vi "Main Page.vi"(8 "error in (no error)":errorcluster, 11 "Node Ptr":T11 format="%.0x") -> (0 "error out":errorcluster)   [LabVIEW 2020, in "NI Synchronization System Explorer.lvlib"]
uses:
  NI Synchronization System Explorer.lvlib
  <vilib>/NI VeriStand/Custom Device API/Custom Device Item Ref.ctl
  Connection Selection.ctl
  Shared/Routes.ctl
  Shared/Route.ctl
  Pins Tab.ctl
  Shared/Mode.ctl
  Shared/External Pin.ctl
  Shared/Time Reference.ctl
  Time Ref Tab.ctl
  Shared/IRIG Type.ctl
  Shared/Constants.vi
  <vilib>/NI VeriStand/Custom Device API/Get Item Property (Boolean).vi
  sub_EnableDisable Control.vi
  <vilib>/NI VeriStand/Custom Device API/Get Item Property (String).vi
  <vilib>/NI VeriStand/Custom Device API/Get Item Property (U16).vi
  <vilib>/NI VeriStand/Custom Device API/Get Item Property (Double).vi
  <vilib>/NI VeriStand/Custom Device API/Set Item Property (String).vi
  <vilib>/NI VeriStand/Custom Device API/Set Item Property (Boolean).vi
  <vilib>/NI VeriStand/Custom Device API/Set Item Property (Variant).vi
  <vilib>/NI VeriStand/Custom Device API/Set Item Property (U16).vi
  <vilib>/NI VeriStand/Custom Device API/Set Item Property (I32).vi
  <vilib>/NI VeriStand/Custom Device API/Set Item Property (Double).vi
  <vilib>/NI VeriStand/Custom Device API/Custom Device API.lvlib
  Shared/NI Synchronization Shared.lvlib
panel:
  in  "6683H Warning":string
  in  "SyncModule":string caption="Chassis Clock Generation Module"
  in  "SyncModule?":bool
  in  "Settings":T1(tab)
  out "TimeRefTab":T2
  in  "Priority 2":i32 min=0 max=255
  in  "Priority 1":i32 min=0 max=255
  in  "IRIG type":T3=enum."IRIGB AM"
  in  "Start Time":timestamp
  in  "PPSSetTime":bool
  in  "Terminal":string
  in  "Time Reference":T4
  out "Mode Desciption 2":string="When using a time reference other than PXI Chassis Clock, it is recommended to additionally configure that time reference in Measurement and Automation Explorer (MAX) before deployment. Doing so will prevent \"macro\" adjustments to system time while the NI VeriStand engine is running."
  out "Mode Desciption":string
  in  "Mode":T5
  in  "ConSelection":T6 caption="Selection"
  out "Pins tab":T7
  in  "PFI2":bool
  in  "PFI1":bool
  in  "PFI0":bool
  in  "PXI_Trig0":bool
  in  "Route In Pin":T8
  in  "Custom Routes":T9
  in  "StartDelay":u16 caption="Generation Start Delay (s)"
  in  "PhaseOffset":dbl caption="Generation Phase Offset (°)" min=0.0 max=360.0
  in  "timekeeper":string caption="Time-Based Synchronization Module"
  in  "Header":cluster{"Section Name":string}={"Section Name"="NI Synchronization Settings"}
  in  "Description":string
  in  "Name":string
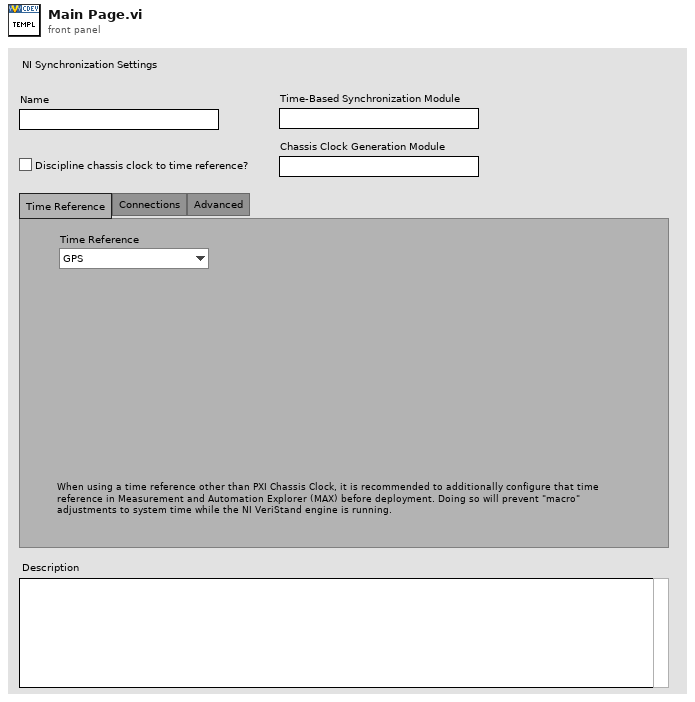
[diagram p1: front panel]
types:
  T1 = enum32{"Time Reference", "Connections", "Advanced"}
  T2 = typedef "NI Synchronization System Explorer.lvlib/Time Ref Tab.ctl" = enum32{"Empty", "1588", "IRIG", "PPS"}
  T3 = typedef "NI Synchronization Shared.lvlib/IRIG Type.ctl" = enum16{"IRIGB DC", "IRIGB AM"}
  T4 = typedef "NI Synchronization Shared.lvlib/Time Reference.ctl" = enum16{"GPS", "IRIG", "PPS", "1588 Ordinary Clock", "802.1AS", "PXI Chassis Clock", "Free Running (Internal)"}
  T5 = typedef "NI Synchronization Shared.lvlib/Mode.ctl" = enum16{"Generate sample clock", "Route sample clock out of chassis", "Route sample clock into chassis", "Custom routes"}
  T6 = typedef "NI Synchronization System Explorer.lvlib/Connection Selection.ctl" = enum16{"Automatic", "Custom"}
  T7 = typedef "NI Synchronization System Explorer.lvlib/Pins Tab.ctl" = enum32{"Pins", "Ext. Pin", "Custom"}
  T8 = typedef "NI Synchronization Shared.lvlib/External Pin.ctl" = enum16{"PFI0", "PFI1", "PFI2"}
  T9 = typedef "NI Synchronization Shared.lvlib/Routes.ctl" = T10[]
  T10 = typedef "NI Synchronization Shared.lvlib/Route.ctl" = cluster{"Source":string, "Destination":string}
  T11 = typedef "Custom Device API.lvlib/Custom Device Item Ref.ctl" = u64
  T12 = typedef "NI Synchronization Shared.lvlib/Connection Settings.ctl" = cluster{"Mode":T5, "pxitrig":bool, "pfi0":bool, "pfi1":bool, "pfi2":bool, "External Pin":T8, "Routes":T9}
  T13 = typedef "Custom Device API.lvlib/Custom Device Item Info.ctl" = cluster{"Name":string, "Is Channel":bool, "GUID":string, "Is Waveform":bool}
  T14 = typedef "NI Synchronization Shared.lvlib/Time Ref Settings.ctl" = cluster{"Time Reference":T4, "Priority 1":i32, "Priority 2":i32, "IRIG type":T3, "Terminal":string, "PPSSetTime":bool, "Start Time":timestamp}
  T15 = typedef "Custom Device API.lvlib/Custom Device Commands.ctl" = enum16{"Default", "Item renamed", "Shutdown", "Dynamic button pressed"}
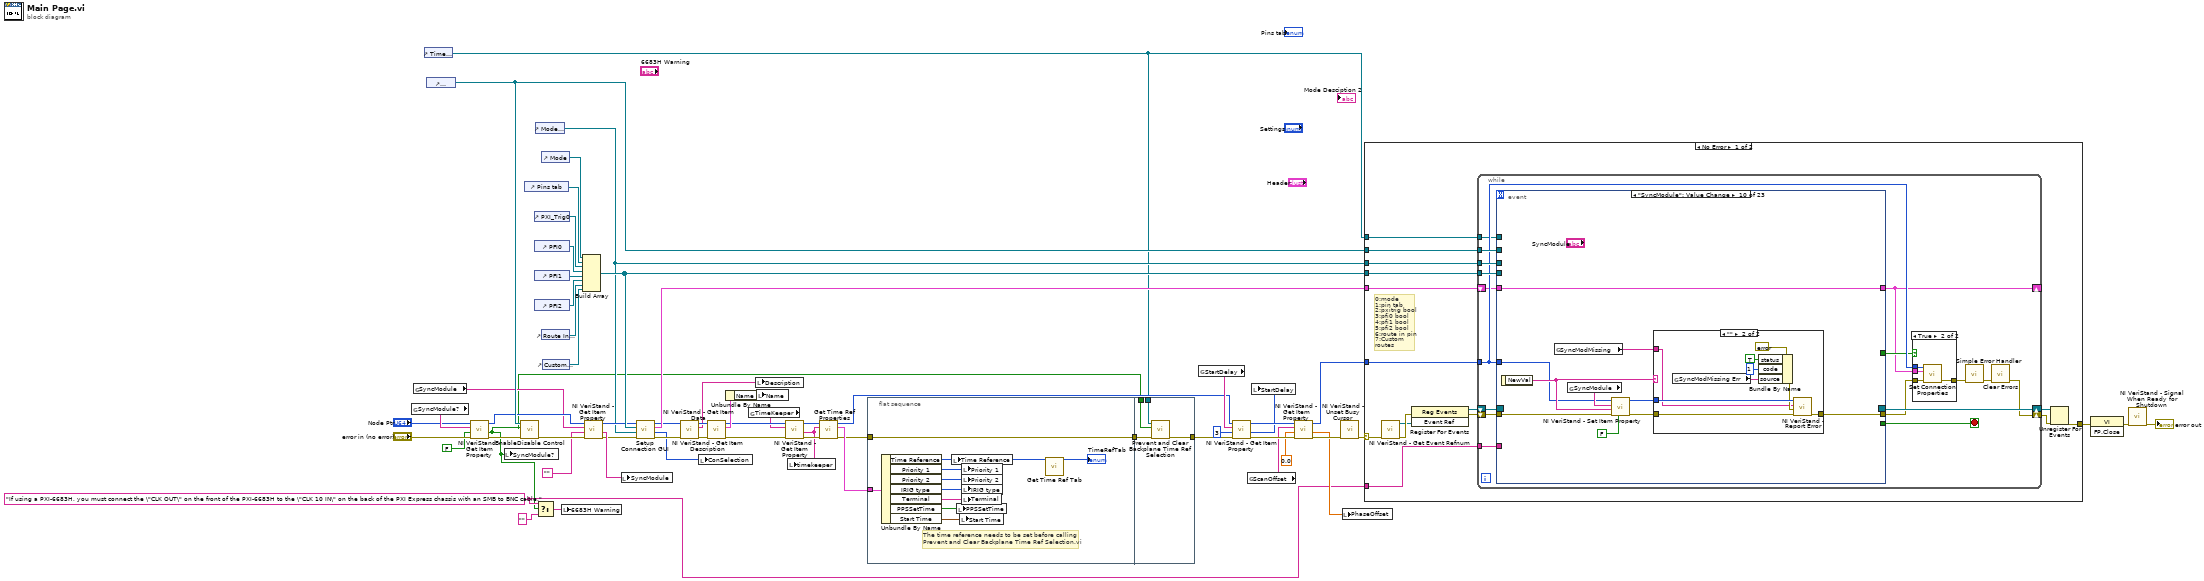
[diagram p0: block diagram]
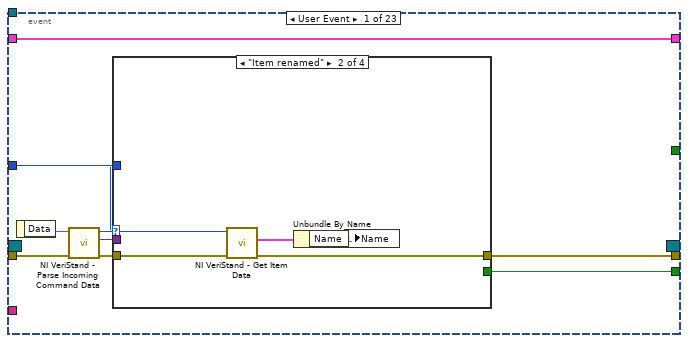
[diagram p3: hidden frame]
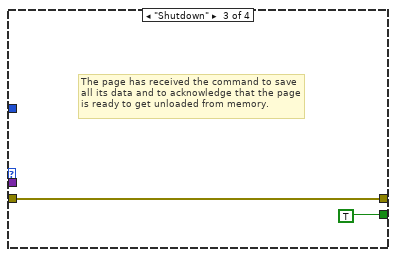
[diagram p5: hidden frame]
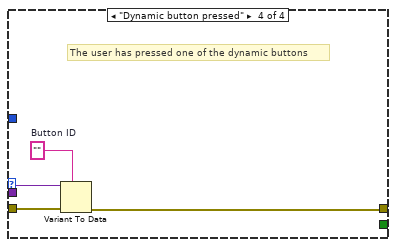
[diagram p6: hidden frame]
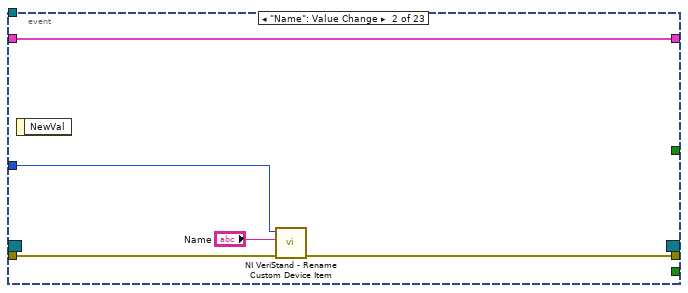
[diagram p7: hidden frame]
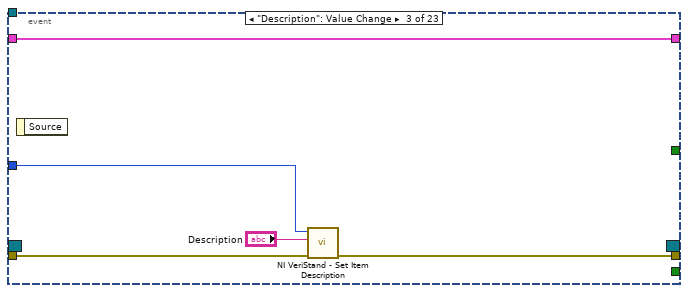
[diagram p8: hidden frame]
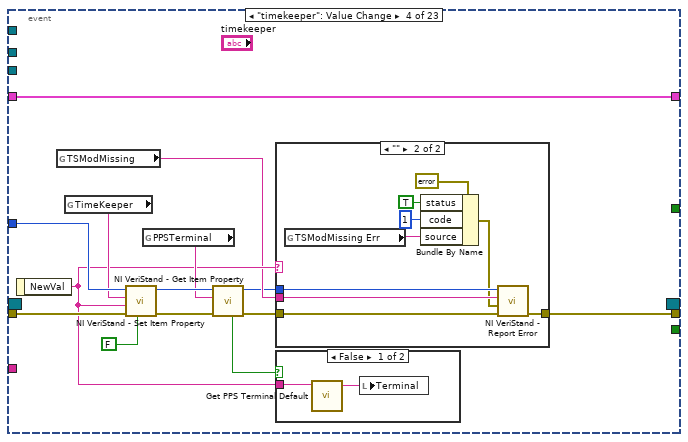
[diagram p9: hidden frame]
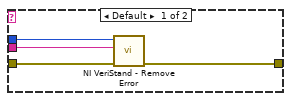
[diagram p10: hidden frame]
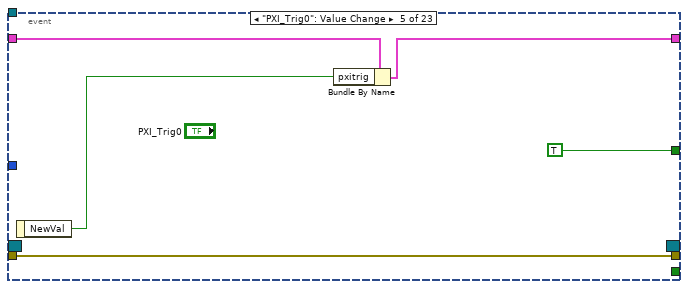
[diagram p12: hidden frame]
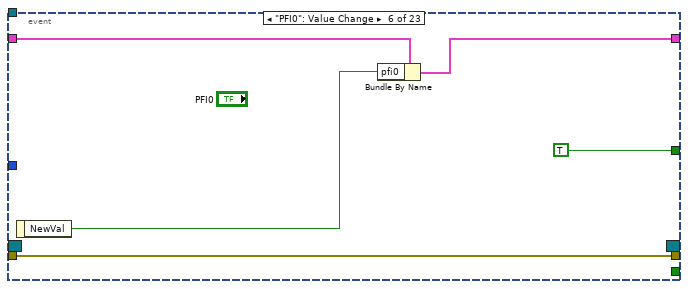
[diagram p13: hidden frame]
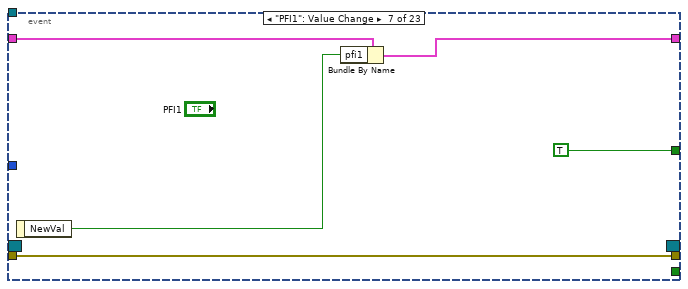
[diagram p14: hidden frame]
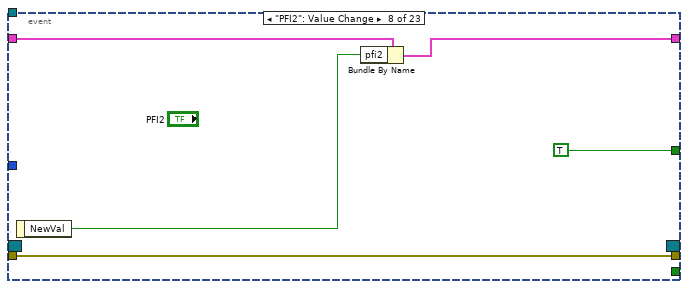
[diagram p15: hidden frame]
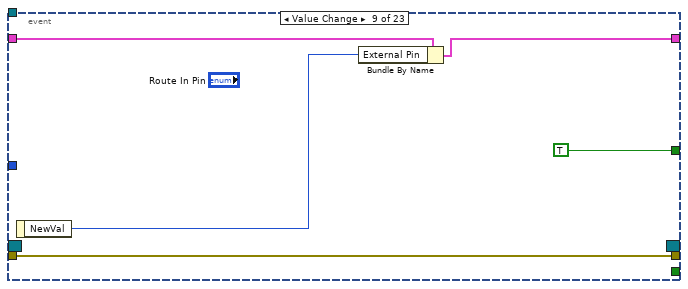
[diagram p16: hidden frame]
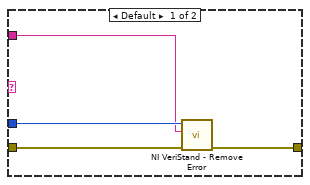
[diagram p17: hidden frame]
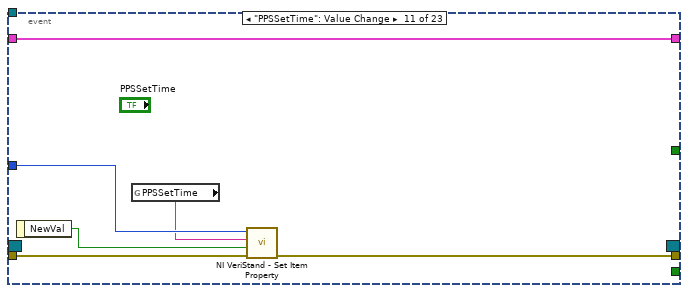
[diagram p18: hidden frame]
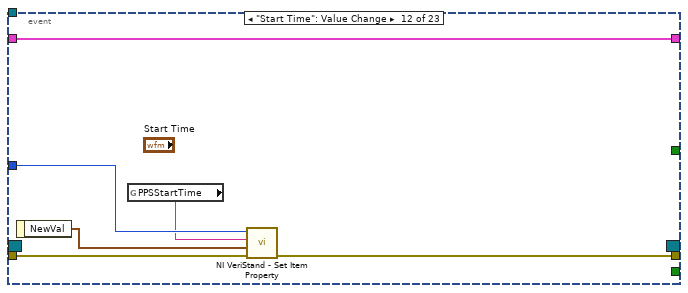
[diagram p19: hidden frame]
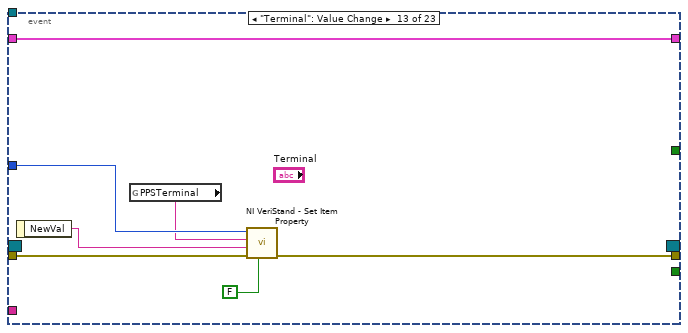
[diagram p20: hidden frame]
diagram:
  w7 = "If using a PXI-6683H, you must connect the \"CLK OUT\" on the front of the PXI-6683H to the \"CLK 10 IN\" on the back of the PXI Express chassis with an SMB to BNC cable." ("6683H Warning")
  n1 = global read "Constants.vi" "SyncModule?"() -> (w27:string)
  n2 = global read "Constants.vi" "SyncModule"() -> (w22:string)
  n3 = control-ref of="Time Reference"() -> (w2:refnum<vi>)
  n4 = control-ref of="SyncModule"() -> (w24:refnum<vi>)
  n5 = call-poly <vilib>:"NI VeriStand - Get Item Property.vi"("error in (no error)"="error in (no error)", "Default Value"=FALSE, "Property Name"=w27, "Item Ref in"="Node Ptr") -> ("error out"=w28:errorcluster, "Value"=w1:bool, "Item Ref out"=w23:T11)  [unwired: 4 in, 1 out]
  n6 = local write "SyncModule?"(w1) -> ()
  n7 = call-poly "EnableDisable Control.vi"("error in (no error)"=w28, "Enable"=w1, "Control"=w24) -> ("error out"=w25:errorcluster)  [unwired: 8 in]
  n8 = control-ref of="Pins tab"() -> (w38:refnum<vi>)
  n9 = control-ref of="PXI_Trig0"() -> (w37:refnum<vi>)
  n10 = control-ref of="PFI0"() -> (w36:refnum<vi>)
  n11 = control-ref of="PFI1"() -> (w31:refnum<vi>)
  n12 = control-ref of="PFI2"() -> (w32:refnum<vi>)
  n13 = control-ref of="Mode Desciption"() -> (w12:refnum<vi>)
  n14 = Select(t=w7, s=w1, f="" ("6683H Warning")) -> (s? t:f=w8:string)
  n15 = control-ref of="Mode"() -> (w39:refnum<vi>)
  n16 = control-ref of="Route In Pin"() -> (w35:refnum<vi>)
  n17 = control-ref of="Custom Routes"() -> (w34:refnum<vi>)
  n18 = local write "6683H Warning"(w8) -> ()
  n19 = Build Array(w39, w38, w37, w36, w31, w32, w35, w34) -> (w29:refnum<vi>[])
  n20 = call-poly <vilib>:"NI VeriStand - Get Item Property.vi"("error in (no error)"=w25, "Default Value"="", "Property Name"=w22, "Item Ref in"=w23) -> ("error out"=w10:errorcluster, "Value"=w20:string, "Item Ref out"=w13:T11)  [unwired: 4 in, 1 out]
  n21 = local write "SyncModule"(w20) -> ()
  n22 = call "Setup Connection GUI.vi"("error in (no error)"=w10, "Mode Description Control"=w12, "Connection Controls"=w29, "Item Ref in"=w13) -> ("error out"=w30:errorcluster, "ConSelection"=w16:T6, "Connection Settings"=w15:T12, "Item Ref out"=w14:T11)  [unwired: 4 in]
  n23 = call <vilib>:"NI VeriStand - Get Item Description.vi"("error in (no error)"=w30, "Item Ref in"=w14) -> ("error out"=w56:errorcluster, "Description"=w57:string, "Item Ref out"=w58:T11)  [unwired: 7 out]
  n24 = local write "ConSelection"(w16) -> ()
  n25 = call <vilib>:"NI VeriStand - Get Item Data.vi"("error in (no error)"=w56, "Item Ref in"=w58) -> ("error out"=w53:errorcluster, "Item Info"=w55:T13, "Item Ref out"=w52:T11)  [unwired: 7 out]
  n26 = Unbundle By Name(w55) -> ("Name"=w54:string)
  n27 = global read "Constants.vi" "TimeKeeper"() -> (w51:string)
  n28 = local write "Description"(w57) -> ()
  n29 = local write "Name"(w54) -> ()
  n30 = call-poly <vilib>:"NI VeriStand - Get Item Property.vi"("error in (no error)"=w53, "Property Name"=w51, "Item Ref in"=w52) -> ("error out"=w50:errorcluster, "Value"=w18:string, "Item Ref out"=w19:T11)  [unwired: 5 in, 1 out]
  n31 = local write "timekeeper"(w18) -> ()
  n32 = call "Get Time Ref Properties.vi"("error in (no error)"=w50, "TimeKeeper Module"=w18, "Device Item Ref in"=w19) -> ("error out"=w6:errorcluster, "Time Ref Settings"=w17:T14, "Item Ref out"=w4:T11)  [unwired: 6 in]
  n33 = flat-sequence {
    tunnel: w17 -> [w72]
    tunnel: w6 -> [w63]
    tunnel: [w63] -> w3
    tunnel: [w75] -> w5
    tunnel: w3 -> [w76]
    tunnel: w2 -> [w74]
    tunnel: w1 -> [w73]
    frame #0 {
      # "The time reference needs to be set before calling \nPrevent and Clear Backplane Time Ref Selection.vi"
      n34 = Unbundle By Name(w72) -> ("Time Reference"=w65:T4, "Priority 1"=w71:i32, "Priority 2"=w70:i32, "IRIG type"=w69:T3, "Terminal"=w68:string, "PPSSetTime"=w67:bool, "Start Time"=w66:timestamp)
      n35 = local write "Time Reference"(w65) -> ()
      n36 = local write "PPSSetTime"(w67) -> ()
      n37 = local write "Start Time"(w66) -> ()
      n38 = local write "Priority 1"(w71) -> ()
      n39 = local write "Priority 2"(w70) -> ()
      n40 = local write "IRIG type"(w69) -> ()
      n41 = local write "Terminal"(w68) -> ()
      n42 = call "Get Time Ref Tab.vi"("Time Ref"=w65) -> ("TimeRefTab"=→"TimeRefTab":T2)  [unwired: 10 in]
    }
    frame #1 {
      n43 = call "Prevent and Clear Backplane Time Ref Selection.vi"("error in (no error)"=w76, "Sync Mod?"=w73, "Time Reference Enum"=w74) -> ("error out"=w75:errorcluster)  [unwired: 8 in]
    }
  }
  n44 = global read "Constants.vi" "StartDelay"() -> (w45:string)
  n45 = call-poly <vilib>:"NI VeriStand - Get Item Property.vi"("error in (no error)"=w5, "Default Value"=u16 3 ("Start Offset Multiple"), "Property Name"=w45, "Item Ref in"=w4) -> ("error out"=w46:errorcluster, "Value"=w43:u16, "Item Ref out"=w49:T11)  [unwired: 4 in, 1 out]
  n46 = global read "Constants.vi" "ScanOffset"() -> (w42:string)
  n47 = local write "StartDelay"(w43) -> ()
  n48 = call-poly <vilib>:"NI VeriStand - Get Item Property.vi"("error in (no error)"=w46, "Default Value"=0.0 ("Scan Offset Scale (%)"), "Property Name"=w42, "Item Ref in"=w49) -> ("error out"=w47:errorcluster, "Value"=w40:dbl, "Item Ref out"=w48:T11)  [unwired: 4 in, 1 out]
  n49 = call <vilib>:"NI VeriStand - Unset Busy Cursor.vi"("error in (no error)"=w47) -> ("error out"=w59:errorcluster)  [unwired: 10 out]
  n50 = local write "PhaseOffset"(w40) -> ()
  n51 = case shown="No Error" w59 {
    selector: w59 -> [w83 w357]
    tunnel: [w88 w355] -> w62
    tunnel: w48 -> [w84 _]
    tunnel: w29 -> [w82 _]
    tunnel: w12 -> [w81 _]
    tunnel: w24 -> [w80 _]
    tunnel: w15 -> [w79 _]
    tunnel: w2 -> [w78 _]
    tunnel: w7 -> [w77 _]
    frame No Error {
      # "0:mode\n1:pin tab\n2:pxitrig bool\n3:pfi0 bool\n4:pfi1 bool\n5:pfi2 bool\n6:route in pin\n7:Custom routes"
      n52 = call <vilib>:"NI VeriStand - Get Event Refnum.vi"("error in (no error)"=w83) -> ("error out"=w91:errorcluster, "Event Ref"=w87:refnum<user-event>)  [unwired: 9 out]
      n53 = register-events(error in=w91, w87) -> (reference out=w85:refnum<event-registration>, error out=w86:errorcluster)  [unwired: 1 in]
      n54 = while {
        tunnel: w84 -> [w97]
        shift-right: [w103] -> w89
        shift-left: w86 -> [w107]
        shift-right: [w108] -> w90
        shift-left: w85 -> [w106]
        tunnel: w82 -> [w102]
        tunnel: w81 -> [w101]
        tunnel: w80 -> [w100]
        shift-right: [w93] -> _
        shift-left: w79 -> [w96]
        tunnel: w78 -> [w94]
        tunnel: w77 -> [w92]
        stop <- w105 stop-if-true
        n55 = event shown="[9] \"SyncModule\": Value Change" {
          selector: w106 -> [_ _ _ _ _ _ _ _ _ _ _ _ _ _ _ _ _ _ _ _ _ _ _]
          dyn-events: [_ _ _ _ _ _ _ _ _ _ _ _ _ _ _ _ _ _ _ _ _ _ _] -> w108
          timeout: _ -> [_ _ _ _ _ _ _ _ _ _ _ _ _ _ _ _ _ _ _ _ _ _ _]
          tunnel: w107 -> [w122 w139 w143 w158 w178 w183 w188 w193 w198 w208 w227 w233 w240 w247 w253 w259 w265 w284 w302 w308 w314 w327 w350]
          tunnel: [w118 _ _ _ _ _ _ _ _ _ _ _ _ _ _ _ _ _ _ _ _ _ _] -> w105
          tunnel: [w117 w138 w142 w147 w178 w183 w188 w193 w198 w201 w223 w229 w236 w244 w249 w255 w261 w272 w302 w304 w310 w322 w347] -> w98
          tunnel: w97 -> [w116 w137 w144 w157 _ _ _ _ _ w199 w226 w232 w239 w246 w252 w258 w264 w277 _ w307 w313 w326 _]
          tunnel: w102 -> [_ _ _ _ _ _ _ _ _ _ _ _ _ _ _ _ _ _ _ _ _ w324 w348]
          tunnel: w101 -> [_ _ _ _ _ _ _ _ _ _ _ _ _ _ _ _ _ _ _ _ _ w323 _]
          tunnel: w100 -> [_ _ _ _ _ _ _ _ _ _ _ _ _ _ _ _ _ w281 _ _ _ _ _]
          tunnel: [w114 w135 w140 w155 w175 w181 w186 w191 w196 w206 w222 w228 w235 w243 w248 w254 w260 w280 w300 w303 w309 w315 w336] -> w93
          tunnel: w96 -> [w114 w135 w140 w155 w176 w182 w187 w192 w197 w206 w222 w228 w235 w243 w248 w254 w260 w280 w301 w303 w309 w317 w337]
          tunnel: [_ _ _ _ TRUE TRUE TRUE TRUE TRUE _ _ _ _ _ _ _ _ _ TRUE _ _ _ TRUE] -> w95
          tunnel: w94 -> [_ _ _ _ _ _ _ _ _ _ _ _ _ _ _ _ _ w279 _ _ _ _ _]
          tunnel: w92 -> [_ _ _ _ _ _ _ _ _ _ _ _ _ _ _ _ _ w276 _ _ _ _ _]
          event User Event {
            n56 = event-data() -> ("Data"=w121:string)  [unwired: 1 out]
            n57 = call <vilib>:"NI VeriStand - Parse Incoming Command Data.vi"("error in (no error)"=w122, "Incoming data"=w121) -> ("error out"=w120:errorcluster, "Outgoing data"=w115:variant, "Action"=w119:T15)  [unwired: 7 out]
            n58 = case shown="\"Item renamed\"" w119 {
              tunnel: w120 -> [w123 w128 w129 w134]
              tunnel: [_ _ TRUE _] -> w118
              tunnel: [w123 w125 w129 w131] -> w117
              tunnel: w116 -> [_ w127 _ _]
              tunnel: w115 -> [_ _ _ w133]
              frame "Default", Default {
              }
              frame "Item renamed" {
                n59 = call <vilib>:"NI VeriStand - Get Item Data.vi"("error in (no error)"=w128, "Item Ref in"=w127) -> ("error out"=w125:errorcluster, "Item Info"=w126:T13)  [unwired: 8 out]
                n60 = Unbundle By Name(w126) -> ("Name"=w124:string)
                n61 = local write "Name"(w124) -> ()
              }
              frame "Shutdown" {
                # "The page has received the command to save all its data and to acknowledge that the page is ready to get unloaded from memory."
              }
              frame "Dynamic button pressed" {
                w132 = ""  # Button ID
                # "The user has pressed one of the dynamic buttons"
                n62 = Variant To Data(error in=w134, type=w132, Variant=w133) -> (error out=w131:errorcluster)  [unwired: 1 out]
              }
            }
          }
          event "Name": Value Change {
            n63 = event-data() -> ()  [unwired: 2 out]
            n64 = call <vilib>:"NI VeriStand - Rename Custom Device Item.vi"("error in (no error)"=w139, "New Name"="Name", "Item Ref in"=w137) -> ("error out"=w138:errorcluster)  [unwired: 1 in, 7 out]
          }
          event "Description": Value Change {
            n65 = event-data() -> ()  [unwired: 2 out]
            n66 = call <vilib>:"NI VeriStand - Set Item Description.vi"("error in (no error)"=w143, "Description"="Description", "Item Ref in"=w144) -> ("error out"=w142:errorcluster)  [unwired: 8 out]
          }
          event "timekeeper": Value Change {
            n67 = event-data() -> ("NewVal"=w148:string)  [unwired: 1 out]
            n68 = global read "Constants.vi" "TSModMissing"() -> (w146:string)
            n69 = global read "Constants.vi" "TimeKeeper"() -> (w156:string)
            n70 = call-poly <vilib>:"NI VeriStand - Set Item Property.vi"("Binary String (T)"=FALSE, "error in (no error)"=w158, "Value"=w148, "Property Name"=w156, "Item Ref in"=w157) -> ("error out"=w153:errorcluster, "Item Ref out"=w152:T11)  [unwired: 4 in, 1 out]
            n71 = global read "Constants.vi" "PPSTerminal"() -> (w151:string)
            n72 = call-poly <vilib>:"NI VeriStand - Get Item Property.vi"("error in (no error)"=w153, "Property Name"=w151, "Item Ref in"=w152) -> ("error out"=w149:errorcluster, "Item Ref out"=w145:T11, "Found?"=w150:bool)  [unwired: 5 in, 1 out]
            n73 = case shown="\"\"" w148 {
              tunnel: w149 -> [w162 w171]
              tunnel: [w159 w170] -> w147
              tunnel: w146 -> [w161 w169]
              tunnel: w145 -> [w160 w168]
              frame Default {
                n74 = call <vilib>:"NI VeriStand - Remove Error.vi"("error in (no error)"=w162, "Error ID"=w161, "Node Ref in"=w160) -> ("error out"=w159:errorcluster)  [unwired: 7 in, 1 out]
              }
              frame "" {
                n75 = global read "Constants.vi" "TSModMissing Err"() -> (w164:string)
                n76 = Bundle By Name(cluster=errorcluster {"status"=FALSE, "code"=0, "source"=""} ("error constant"), "status"=TRUE, "code"=1, "source"=w164) -> (w163:errorcluster)
                n77 = call <vilib>:"NI VeriStand - Report Error.vi"("error in (no error)"=w171, "New Error"=w163, "Error ID"=w169, "Node Ref in"=w168) -> ("error out"=w170:errorcluster)  [unwired: 6 in, 1 out]
              }
            }
            n78 = case shown="False" w150 {
              tunnel: w148 -> [w173 _]
              frame False {
                n79 = call "Get PPS Terminal Default.vi"("TimeKeeper Module"=w173) -> ("PPSTerminal Default"=w172:string)  [unwired: 10 in]
                n80 = local write "Terminal"(w172) -> ()
              }
              frame True {
              }
            }
          }
          event "PXI_Trig0": Value Change {
            n81 = event-data() -> ("NewVal"=w177:bool)  [unwired: 1 out]
            n82 = Bundle By Name(cluster=w176, "pxitrig"=w177) -> (w175:T12)
          }
          event "PFI0": Value Change {
            n83 = event-data() -> ("NewVal"=w180:bool)  [unwired: 1 out]
            n84 = Bundle By Name(cluster=w182, "pfi0"=w180) -> (w181:T12)
          }
          event "PFI1": Value Change {
            n85 = event-data() -> ("NewVal"=w185:bool)  [unwired: 1 out]
            n86 = Bundle By Name(cluster=w187, "pfi1"=w185) -> (w186:T12)
          }
          event "PFI2": Value Change {
            n87 = event-data() -> ("NewVal"=w190:bool)  [unwired: 1 out]
            n88 = Bundle By Name(cluster=w192, "pfi2"=w190) -> (w191:T12)
          }
          event Value Change {
            n89 = event-data() -> ("NewVal"=w195:T8)  [unwired: 1 out]
            n90 = Bundle By Name(cluster=w197, "External Pin"=w195) -> (w196:T12)
          }
          event "SyncModule": Value Change {
            n91 = event-data() -> ("NewVal"=w203:string)  [unwired: 1 out]
            n92 = global read "Constants.vi" "SyncModMissing"() -> (w200:string)
            n93 = global read "Constants.vi" "SyncModule"() -> (w207:string)
            n94 = call-poly <vilib>:"NI VeriStand - Set Item Property.vi"("Binary String (T)"=FALSE, "error in (no error)"=w208, "Value"=w203, "Property Name"=w207, "Item Ref in"=w199) -> ("error out"=w202:errorcluster, "Item Ref out"=w204:T11)  [unwired: 4 in, 1 out]
            n95 = case shown="\"\"" w203 {
              tunnel: w202 -> [w212 w221]
              tunnel: [w210 w220] -> w201
              tunnel: w204 -> [w211 w219]
              tunnel: w200 -> [w209 w213]
              frame Default {
                n96 = call <vilib>:"NI VeriStand - Remove Error.vi"("error in (no error)"=w212, "Error ID"=w209, "Node Ref in"=w211) -> ("error out"=w210:errorcluster)  [unwired: 7 in, 1 out]
              }
              frame "" {
                n97 = global read "Constants.vi" "SyncModMissing Err"() -> (w214:string)
                n98 = Bundle By Name(cluster=errorcluster {"status"=FALSE, "code"=0, "source"=""} ("error constant"), "status"=TRUE, "code"=1, "source"=w214) -> (w215:errorcluster)
                n99 = call <vilib>:"NI VeriStand - Report Error.vi"("error in (no error)"=w221, "New Error"=w215, "Error ID"=w213, "Node Ref in"=w219) -> ("error out"=w220:errorcluster)  [unwired: 6 in, 1 out]
              }
            }
          }
          event "PPSSetTime": Value Change {
            n100 = event-data() -> ("NewVal"=w224:bool)  [unwired: 1 out]
            n101 = global read "Constants.vi" "PPSSetTime"() -> (w225:string)
            n102 = call-poly <vilib>:"NI VeriStand - Set Item Property.vi"("error in (no error)"=w227, "Value"=w224, "Property Name"=w225, "Item Ref in"=w226) -> ("error out"=w223:errorcluster)  [unwired: 5 in, 2 out]
          }
          event "Start Time": Value Change {
            n103 = event-data() -> ("NewVal"=w230:timestamp)  [unwired: 1 out]
            n104 = global read "Constants.vi" "PPSStartTime"() -> (w231:string)
            n105 = call-poly <vilib>:"NI VeriStand - Set Item Property.vi"("error in (no error)"=w233, "Value"=w230, "Property Name"=w231, "Item Ref in"=w232) -> ("error out"=w229:errorcluster)  [unwired: 5 in, 2 out]
          }
          event "Terminal": Value Change {
            n106 = event-data() -> ("NewVal"=w237:string)  [unwired: 1 out]
            n107 = global read "Constants.vi" "PPSTerminal"() -> (w238:string)
            n108 = call-poly <vilib>:"NI VeriStand - Set Item Property.vi"("Binary String (T)"=FALSE, "error in (no error)"=w240, "Value"=w237, "Property Name"=w238, "Item Ref in"=w239) -> ("error out"=w236:errorcluster)  [unwired: 4 in, 2 out]
          }
          event Value Change {
            n109 = event-data() -> ("NewVal"=w242:T4)  [unwired: 1 out]
            n110 = call "Get Time Ref Tab.vi"("Time Ref"=w242) -> ("TimeRefTab"=w241:T2)  [unwired: 10 in]
            n111 = global read "Constants.vi" "TimeRef"() -> (w245:string)
            n112 = local write "TimeRefTab"(w241) -> ()
            n113 = call-poly <vilib>:"NI VeriStand - Set Item Property.vi"("error in (no error)"=w247, "Value"=w242, "Property Name"=w245, "Item Ref in"=w246) -> ("error out"=w244:errorcluster)  [unwired: 5 in, 2 out]
          }
          event Value Change {
            n114 = event-data() -> ("NewVal"=w250:T3)  [unwired: 1 out]
            n115 = global read "Constants.vi" "IRIGType"() -> (w251:string)
            n116 = call-poly <vilib>:"NI VeriStand - Set Item Property.vi"("error in (no error)"=w253, "Value"=w250, "Property Name"=w251, "Item Ref in"=w252) -> ("error out"=w249:errorcluster)  [unwired: 5 in, 2 out]
          }
          event "Priority 1": Value Change {
            n117 = event-data() -> ("NewVal"=w256:i32)  [unwired: 1 out]
            n118 = global read "Constants.vi" "Priority1"() -> (w257:string)
            n119 = call-poly <vilib>:"NI VeriStand - Set Item Property.vi"("error in (no error)"=w259, "Value"=w256, "Property Name"=w257, "Item Ref in"=w258) -> ("error out"=w255:errorcluster)  [unwired: 5 in, 2 out]
          }
          event "Priority 2": Value Change {
            n120 = event-data() -> ("NewVal"=w262:i32)  [unwired: 1 out]
            n121 = global read "Constants.vi" "Priority2"() -> (w263:string)
            n122 = call-poly <vilib>:"NI VeriStand - Set Item Property.vi"("error in (no error)"=w265, "Value"=w262, "Property Name"=w263, "Item Ref in"=w264) -> ("error out"=w261:errorcluster)  [unwired: 5 in, 2 out]
          }
          event "SyncModule?": Value Change {
            n123 = event-data() -> ("NewVal"=w268:bool)  [unwired: 1 out]
            n124 = local read "SyncModule"() -> (w270:string)
            n125 = global read "Constants.vi" "SyncModule?"() -> (w283:string)
            n126 = call-poly <vilib>:"NI VeriStand - Set Item Property.vi"("error in (no error)"=w284, "Value"=w268, "Property Name"=w283, "Item Ref in"=w277) -> ("error out"=w282:errorcluster, "Item Ref out"=w271:T11)  [unwired: 5 in, 1 out]
            n127 = Select(t=w276, s=w268, f="") -> (s? t:f=w274:string)
            n128 = Empty String/Path?(string/path=w270) -> (empty?=w269:bool)
            n129 = call-poly "EnableDisable Control.vi"("error in (no error)"=w282, "Enable"=w268, "Control"=w281) -> ("error out"=w278:errorcluster)  [unwired: 8 in]
            n130 = local write "6683H Warning"(w274) -> ()
            n131 = call "Prevent and Clear Backplane Time Ref Selection.vi"("error in (no error)"=w278, "Sync Mod?"=w268, "Time Reference Enum"=w279) -> ("error out"=w273:errorcluster)  [unwired: 8 in]
            n132 = And(x=w269, y=w268) -> (x .and. y?=w267:bool)
            n133 = global read "Constants.vi" "SyncModMissing"() -> (w266:string)
            n134 = case shown="True" w267 {
              tunnel: w273 -> [w288 w296]
              tunnel: [w287 w297] -> w272
              tunnel: w271 -> [w286 w295]
              tunnel: w266 -> [w285 w290]
              frame False {
                # "syncModule disabled\nclear errors due to empty device string"
                n135 = call <vilib>:"NI VeriStand - Remove Error.vi"("error in (no error)"=w288, "Error ID"=w285, "Node Ref in"=w286) -> ("error out"=w287:errorcluster)  [unwired: 7 in, 1 out]
              }
              frame True {
                # "syncModule enabled\nbut SyncModule string is empty\nset error"
                n136 = global read "Constants.vi" "SyncModMissing Err"() -> (w289:string)
                n137 = Bundle By Name(cluster=errorcluster {"status"=FALSE, "code"=0, "source"=""} ("error constant"), "status"=TRUE, "code"=1, "source"=w289) -> (w291:errorcluster)
                n138 = call <vilib>:"NI VeriStand - Report Error.vi"("error in (no error)"=w296, "New Error"=w291, "Error ID"=w290, "Node Ref in"=w295) -> ("error out"=w297:errorcluster)  [unwired: 6 in, 1 out]
              }
            }
          }
          event Value Change {
            n139 = event-data() -> ("NewVal"=w299:T9)  [unwired: 1 out]
            n140 = Bundle By Name(cluster=w301, "Routes"=w299) -> (w300:T12)
          }
          event "PhaseOffset": Value Change {
            n141 = event-data() -> ("NewVal"=w305:dbl)  [unwired: 1 out]
            n142 = global read "Constants.vi" "ScanOffset"() -> (w306:string)
            n143 = call-poly <vilib>:"NI VeriStand - Set Item Property.vi"("error in (no error)"=w308, "Value"=w305, "Property Name"=w306, "Item Ref in"=w307) -> ("error out"=w304:errorcluster)  [unwired: 5 in, 2 out]
          }
          event "StartDelay": Value Change {
            n144 = event-data() -> ("NewVal"=w311:u16)  [unwired: 1 out]
            n145 = global read "Constants.vi" "StartDelay"() -> (w312:string)
            n146 = call-poly <vilib>:"NI VeriStand - Set Item Property.vi"("error in (no error)"=w314, "Value"=w311, "Property Name"=w312, "Item Ref in"=w313) -> ("error out"=w310:errorcluster)  [unwired: 5 in, 2 out]
          }
          event Value Change {
            n147 = event-data() -> ("NewVal"=w320:T6)  [unwired: 1 out]
            n148 = global read "Constants.vi" "ConSelection"() -> (w325:string)
            n149 = call-poly <vilib>:"NI VeriStand - Set Item Property.vi"("error in (no error)"=w327, "Value"=w320, "Property Name"=w325, "Item Ref in"=w326) -> ("error out"=w321:errorcluster, "Item Ref out"=w318:T11)  [unwired: 5 in, 1 out]
            n150 = case shown="\"Custom\"" w320 {
              tunnel: w321 -> [w329 w334]
              tunnel: [w329 w333] -> w319
              tunnel: w318 -> [w328 w332]
              tunnel: w317 -> [_ w331]
              tunnel: [w328 w330] -> w316
              frame "Automatic" {
              }
              frame "Custom" {
                n151 = call "Set Connection Properties.vi"("error in (no error)"=w334, "AutoSelect"=w331, "Device Item Ref in"=w332) -> ("error out"=w333:errorcluster, "Item Ref out"=w330:T11)  [unwired: 7 in]
              }
            }
            n152 = call "Setup Connection GUI.vi"("error in (no error)"=w319, "Mode Description Control"=w323, "Connection Controls"=w324, "Item Ref in"=w316) -> ("error out"=w322:errorcluster, "Connection Settings"=w315:T12)  [unwired: 4 in, 2 out]
          }
          event Value Change {
            n153 = event-data() -> ("NewVal"=w340:T5)  [unwired: 1 out]
            n154 = Equal?(x=w340, y=Mode."Route sample clock out of chassis" ("x")) -> (x = y?=w338:bool)
            n155 = Equal?(x=w340, y=Mode."Generate sample clock" ("x")) -> (x = y?=w342:bool)
            n156 = Index Array(array=w348, index=2) -> (element=w344:refnum<vi>)
            n157 = call "Get Connection Description Text and Pins Tab.vi"("Mode"=w340) -> ("Pins tab"=w346:T7, "Description"=→"Mode Desciption":string)  [unwired: 9 in]
            n158 = local write "Pins tab"(w346) -> ()
            n159 = call-poly "EnableDisable Control.vi"("error in (no error)"=w350, "Enable"=w342, "Control"=w344) -> ("error out"=w347:errorcluster)  [unwired: 8 in]
            n160 = Bundle By Name(cluster=w337, "Mode"=w340) -> (w335:T12)
            n161 = case shown="True" w338 {
              tunnel: w335 -> [w351 w354]
              tunnel: [w351 w353] -> w336
              frame False {
              }
              frame True {
                n162 = Bundle By Name(cluster=w354, "pxitrig"=FALSE) -> (w353:T12)
              }
            }
          }
        }
        n163 = case shown="True" w95 {
          tunnel: [w109 w113] -> w99
          tunnel: w98 -> [w109 w112]
          tunnel: w97 -> [_ w111]
          tunnel: w93 -> [_ w110]
          frame False {
          }
          frame True {
            n164 = call "Set Connection Properties.vi"("error in (no error)"=w112, "AutoSelect"=w110, "Device Item Ref in"=w111) -> ("error out"=w113:errorcluster)  [unwired: 7 in, 1 out]
          }
        }
        n165 = call <vilib>:"Simple Error Handler.vi"("error in (no error)"=w99) -> ("error out"=w104:errorcluster)  [unwired: 1 in, 7 out]
        n166 = call <vilib>:"Clear Errors.vi"("error in (no error)"=w104) -> ("error out"=w103:errorcluster)  [unwired: 1 in, 5 out]
      }
      n167 = Unregister For Events(event registration refnum=w90, error in=w89) -> (error out=w88:errorcluster)
    }
    frame Error {
      n168 = call <vilib>:"Simple Error Handler.vi"("error in (no error)"=w357) -> ("error out"=w356:errorcluster)  [unwired: 1 in, 7 out]
      n169 = call <vilib>:"Clear Errors.vi"("error in (no error)"=w356) -> ("error out"=w355:errorcluster)  [unwired: 1 in, 5 out]
    }
  }
  n170 = invoke class="VI" method="FP.Close"(error in=w62) -> (error out=w61:errorcluster)  [unwired: 2 in, 2 out]
  n171 = call <vilib>:"NI VeriStand - Signal When Ready for Shutdown.vi"("error in (no error)"=w61) -> ("error out"=→"error out":errorcluster)  [unwired: 10 out]
